vi "New PropertyContainer.vi"(8 "error in (no error)":errorcluster) -> (0 "error out":errorcluster, 3 "Session Handle out":T1)   [LabVIEW 2020, in "TSS.lvlib" / "VariableContainer.lvclass"]
uses:
  VariableContainer.lvclass
  Typedefs/Session Handle.ctl
  Engine/Engine.lvclass
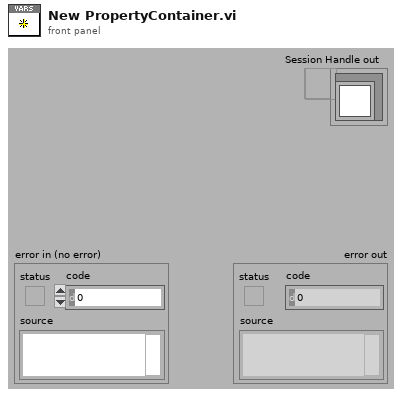
[diagram p1: front panel]
types:
  T1 = typedef "TSS.lvlib/VariableContainer.lvclass/Session Handle.ctl" = refnum<data-value>
  T2 = typedef "TSS.lvlib/Engine.lvclass/Session Handle.ctl" = refnum<data-value>
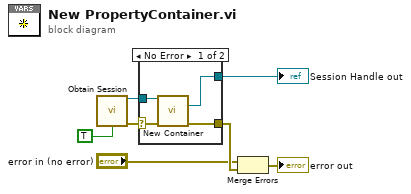
[diagram p0: block diagram]
diagram:
  n1 = call "Obtain Session.vi"("Error to Create? (F)"=TRUE) -> ("Session Handle"=w5:T2, "error out"=w6:errorcluster)  [unwired: 12 in, 1 out]
  n2 = case shown="No Error" w6 {
    selector: w6 -> [w10 w12]
    tunnel: w5 -> [w11 _]
    tunnel: [w9 _] -> w3
    tunnel: [w8 w12] -> w4
    frame No Error {
      n3 = call "New Container.vi"("Session Handle in"=w11, "error in (no error)"=w10) -> ("New Value Container"=w9:T1, "error out"=w8:errorcluster)  [unwired: 11 in, 1 out]
    }
    frame Error {
    }
  }
  "Session Handle out" <- w3
  n4 = Merge Errors("error in (no error)", w4) -> (→"error out":errorcluster)
